vi "Get Generic Slave IOVars.vi"(8 "error in (no error)":errorcluster, 11 "ECAT Slave in":refnum<k21>="ni.var.io://localhost/EtherCAT Master/Device") -> (0 "error IO":errorcluster, 2 "ECAT Variablenobjekt":refnum<k21>[](array[refnum]), 3 "ECAT Slave out":refnum<k21>="ni.var.io:/")   [LabVIEW 2027, in "SEECD Engine.lvlib"]
uses:
  SEECD Engine.lvlib
  <resource>/objmgr/IndComECAT.rc
  <vilib>/NI VeriStand/Custom Device Tools/Custom Device Utility Library/Custom Device Utility Library.lvlib
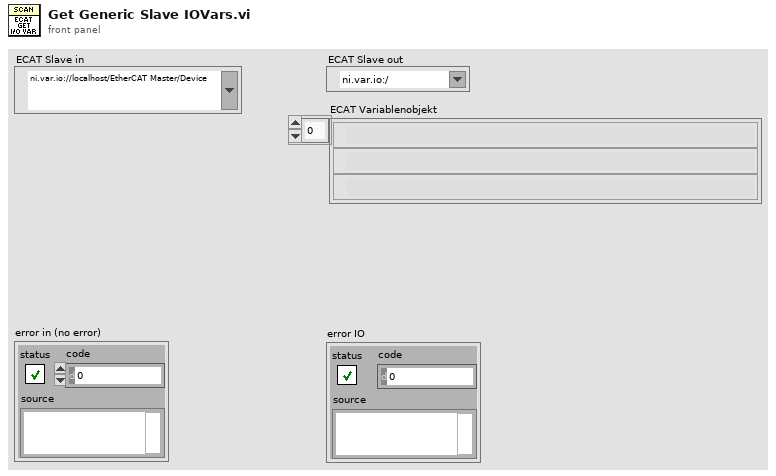
[diagram p1: front panel]
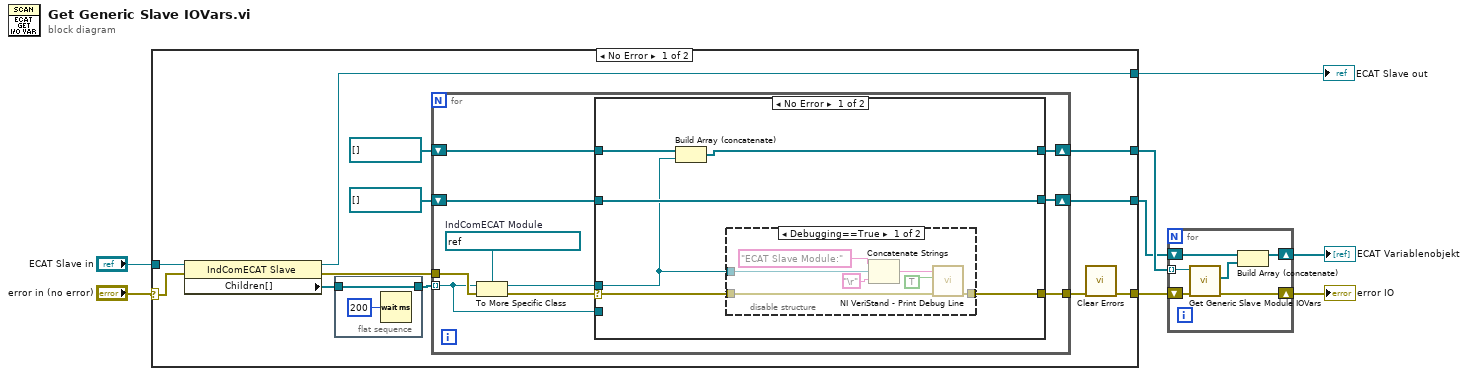
[diagram p0: block diagram]
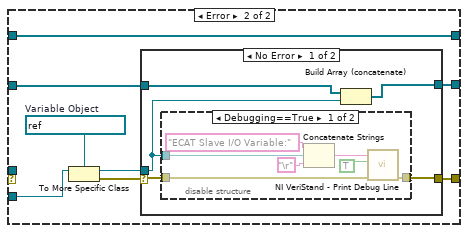
[diagram p3: hidden frame]
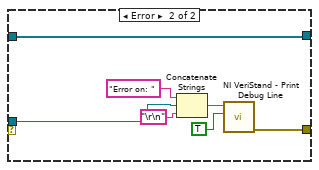
[diagram p5: hidden frame]
diagram:
  n1 = case shown="No Error" "error in (no error)" {
    selector: "error in (no error)" -> [w17 w76]
    tunnel: [w20 w76] -> w5
    tunnel: "ECAT Slave in" -> [w19 w75]
    tunnel: [w18 w75] -> w7
    tunnel: [w11 _] -> w2
    tunnel: [w9 _] -> w3
    frame No Error {
      n2 = property class="IndComECAT Slave"(reference=w19, error in=w17) -> (reference out=w18:refnum<k21>, error out=w16:errorcluster, "Children[]"=w14:refnum<k21>[])
      n3 = flat-sequence {
        tunnel: w14 -> [w22]
        tunnel: [w22] -> w13
        frame #0 {
          n4 = Wait (ms)(milliseconds to wait=u32 200) -> ()  [unwired: 1 out]
        }
      }
      n5 = for {
        tunnel: w13 -> [w23] mode=indexing
        tunnel: w16 -> [w29]
        tunnel: [w32] -> w15
        shift-right: [w31] -> w11
        shift-left: refnum<k21>[] [] -> [w30]
        shift-right: [w25] -> w9
        shift-left: refnum<k21>[] [] -> [w26]
        w28 = refnum<k21> refnum  # IndComECAT Module
        n6 = To More Specific Class(target class=w28, reference=w23, error in=w29) -> (specific class reference=w24:refnum<k21>, error out=w27:errorcluster)
        n7 = case shown="No Error" w27 {
          selector: w27 -> [w35 _]
          tunnel: [w34 w54] -> w32
          tunnel: [w36 w51] -> w31
          tunnel: w30 -> [w36 w50]
          tunnel: w26 -> [w38 w48]
          tunnel: [w37 w48] -> w25
          tunnel: w24 -> [w33 _]
          tunnel: w23 -> [_ w47]
          frame No Error {
            n8 = Build Array (concatenate)(w38, w33) -> (w37:refnum<k21>[])
            n9 = disable-structure shown="Debugging==True" {
              disable-tunnel: w33 -> [w45 _]
              disable-tunnel: [w43 w46] -> w34
              disable-tunnel: w35 -> [w42 w46]
              frame condition #0 {
                n10 = Concatenate Strings("ECAT Slave Module:", w45, "\r") -> (w41:string)
                n11 = call <vilib>:"NI VeriStand - Print Debug Line.vi"("error in (no error)"=w42, "Add to log file? (F)"=TRUE, "Message"=w41) -> ("error out"=w43:errorcluster)  [unwired: 8 in]
              }
              frame condition #1 (active) {
              }
            }
          }
          frame Error {
            w49 = refnum<k21> refnum  # Variable Object
            n12 = To More Specific Class(target class=w49, reference=w47) -> (specific class reference=w52:refnum<k21>, error out=w53:errorcluster)  [unwired: 1 in]
            n13 = case shown="No Error" w53 {
              selector: w53 -> [w55 _]
              tunnel: w52 -> [w57 w69]
              tunnel: [w56 w71] -> w54
              tunnel: [w58 w74] -> w51
              tunnel: w50 -> [w59 w74]
              frame No Error {
                n14 = disable-structure shown="Debugging==True" {
                  disable-tunnel: w57 -> [w66 _]
                  disable-tunnel: [w64 w67] -> w56
                  disable-tunnel: w55 -> [w63 w67]
                  frame condition #0 {
                    n15 = Concatenate Strings("ECAT Slave I/O Variable:", w66, "\r") -> (w62:string)
                    n16 = call <vilib>:"NI VeriStand - Print Debug Line.vi"("error in (no error)"=w63, "Add to log file? (F)"=TRUE, "Message"=w62) -> ("error out"=w64:errorcluster)  [unwired: 8 in]
                  }
                  frame condition #1 (active) {
                  }
                }
                n17 = Build Array (concatenate)(w59, w57) -> (w58:refnum<k21>[])
              }
              frame Error {
                n18 = Concatenate Strings("Error on: ", w69, "\r\n") -> (w72:string)
                n19 = call <vilib>:"NI VeriStand - Print Debug Line.vi"("Add to log file? (F)"=TRUE ("Add to log file? (T)"), "Message"=w72) -> ("error out"=w71:errorcluster)  [unwired: 9 in]
              }
            }
          }
        }
      }
      n20 = call <vilib>:"Clear Errors.vi"("error in (no error)"=w15) -> ("error out"=w20:errorcluster)  [unwired: 5 in, 1 out]
    }
    frame Error {
    }
  }
  "ECAT Slave out" <- w7
  n21 = for {
    shift-right: [w81] -> w4
    shift-left: w5 -> [w82]
    tunnel: w3 -> [w80] mode=indexing
    shift-right: [w79] -> w1
    shift-left: w2 -> [w78]
    n22 = call "Get Generic Slave Module IOVars.vi"("error in (no error)"=w82, "ECAT Slave Module in"=w80) -> ("error IO"=w81:errorcluster, "ECAT Variablenobjekt"=w77:refnum<k21>[])  [unwired: 8 in]
    n23 = Build Array (concatenate)(w78, w77) -> (w79:refnum<k21>[])
  }
  "error IO" <- w4
  "ECAT Variablenobjekt" <- w1
